vi "startTime.get.vi"(8 "error in (no error)":errorcluster, 11 "Run in":refnum<class "Run.lvclass">) -> (0 "error out":errorcluster, 2 "startTime":timestamp format="%<%x %.3X>T", 3 "Run out":refnum<class "Run.lvclass">)   [LabVIEW 2020, in "Run.lvclass"]
uses:
  Run.lvclass
  Run.lvclass/Run.ctl
  20fa2b38-31a7-4466-a6b6-6ae4e02b8116.vi
  a23810a7-3b77-49a4-899b-4f9ad3fa80dd.vi
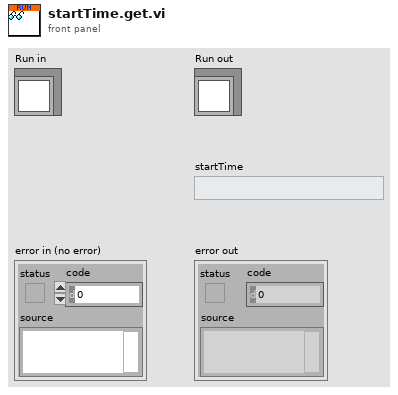
[diagram p1: front panel]
types:
  T1 = cluster{"secondsSinceEpoch":i32, "offsetNanoseconds":i32}
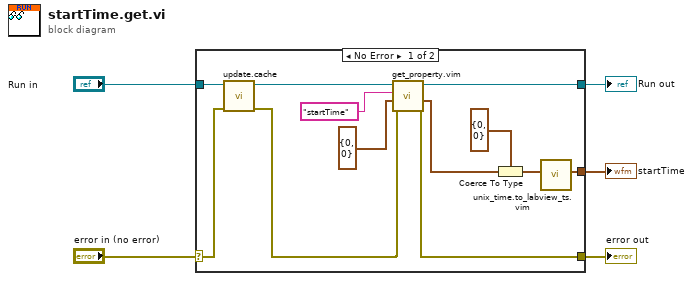
[diagram p0: block diagram]
diagram:
  n1 = case shown="No Error" "error in (no error)" {
    selector: "error in (no error)" -> [w17 w18]
    tunnel: [w8 w18] -> w4
    tunnel: [w6 w19] -> w2
    tunnel: "Run in" -> [w13 w19]
    tunnel: [w16 _] -> w1
    frame No Error {
      n2 = call "update.cache.vi"("error in"=w17, "Run in"=w13) -> ("error out"=w9:errorcluster, "Run out"=w7:refnum<class "Run.lvclass">)  [unwired: 8 in]
      n3 = call "get_property.vim"("error in"=w9, "default value and type"=T1 {"secondsSinceEpoch"=0, "offsetNanoseconds"=0} ("startTime"), "Property Name"="startTime", "Run in"=w7) -> ("error out"=w8:errorcluster, "Value"=w10:T1, "Run out"=w6:refnum<class "Run.lvclass">)  [unwired: 5 in]
      n4 = Coerce To Type(0:w10, 1:cluster{"Seconds":i32, "Nanoseconds":i32} {"Seconds"=0, "Nanoseconds"=0} ("UNIX Timestamp")) -> (2:w14:cluster{"Seconds":i32, "Nanoseconds":i32})
      n5 = call "unix_time.to_labview_ts.vim"("UNIX Timestamp"=w14) -> ("Time Stamp"=w16:timestamp)  [unwired: 10 in]
    }
    frame Error {
    }
  }
  "error out" <- w4
  "Run out" <- w2
  "startTime" <- w1
